vi "test Get-Set-Get Parameter Definitions.vi"(8 "error in":errorcluster, 11 "TestCase in":refnum<class "Scripting.lvclass">) -> (0 "error out":errorcluster, 3 "TestCase out":refnum<class "Scripting.lvclass">)   [LabVIEW 2020, in "Scripting.lvclass"]
uses:
  Scripting.lvclass
  Shared/Parameter Definition.ctl
  <vilib>/NI/NI VeriStand Encoding and Decoding/Encoding.ctl
  Scripting.lvclass/Scripting.ctl
  Scripting/Ballard/Constants.vi
  <vilib>/NI VeriStand/Custom Device Tools/Custom Device Utility Library/NI VeriStand - Search for Item by GUID.vi
  <vilib>/addons/_JKI Toolkits/VI Tester/TestCase.llb/TestCase.lvclass
  Scripting/Ballard/Ballard ARINC 429 Scripting.lvlib
  Scripting/ARINC 429/ARINC 429 Scripting.lvlib
  <vilib>/NI/NI VeriStand Encoding and Decoding/Encoding and Decoding.lvlib
  <vilib>/NI VeriStand/Custom Device Tools/Custom Device Utility Library/Custom Device Utility Library.lvlib
  <vilib>/NI VeriStand/Custom Device API/Custom Device API.lvlib
  C:/Program Files (x86)/National Instruments/LabVIEW 2020/vi.lib/addons/_JKI Toolkits/VI Tester/TestCase.llb/TestCase.lvclass
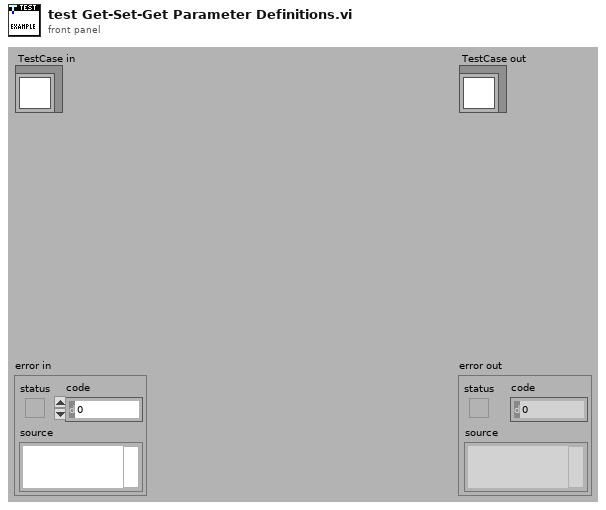
[diagram p1: front panel]
types:
  T1 = typedef "Parameter Definition.ctl" = cluster{"start index":i32, "size":i32, "encoding":T2, "signed":bool, "scale multiplier":dbl, "scale offset":dbl}
  T2 = typedef "Encoding and Decoding.lvlib/Encoding.ctl" = enum16{"BNR", "BCD", "Discrete"}
  T3 = typedef "Custom Device API.lvlib/Custom Device Item Ref.ctl" = u64
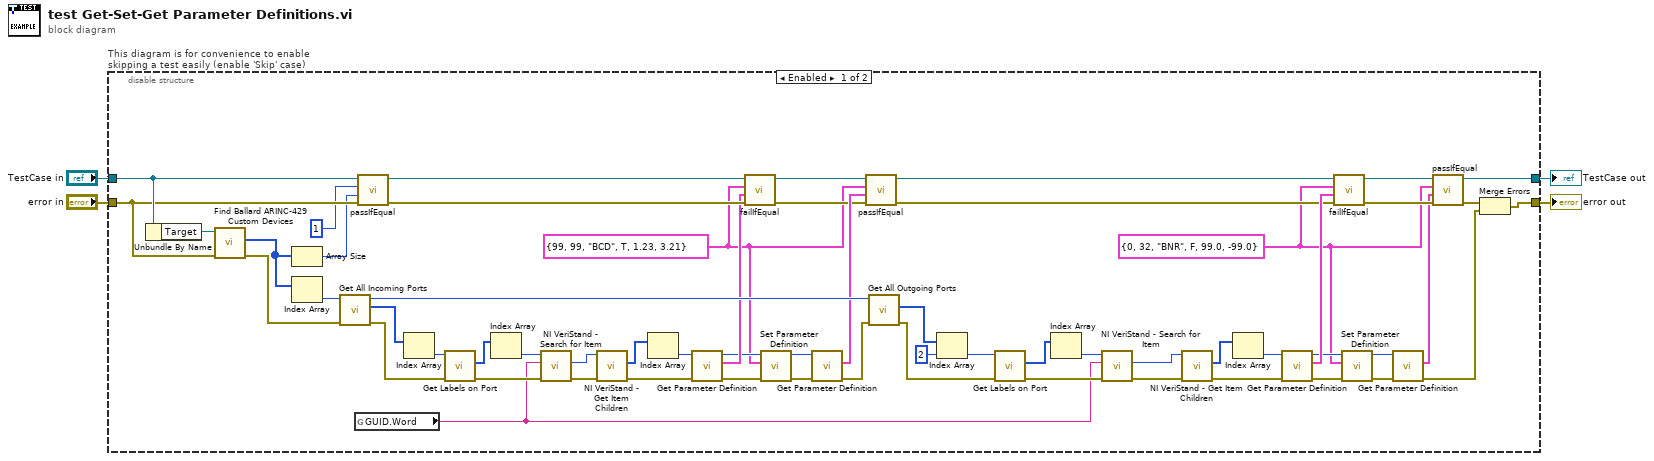
[diagram p0: block diagram]
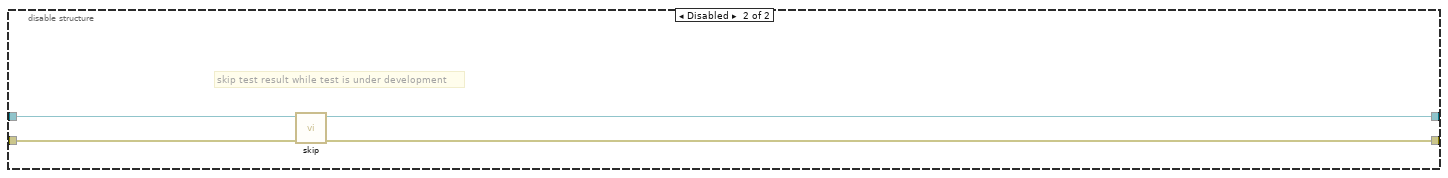
[diagram p2: hidden frame]
diagram:
  n1 = disable-structure "This diagram is for convenience to enable skipping a test easily (enable 'Skip' case)" shown="Enabled" {
    disable-tunnel: "TestCase in" -> [w62 w68]
    disable-tunnel: [w8 w66] -> w1
    disable-tunnel: [w51 w67] -> w3
    disable-tunnel: "error in" -> [w61 w65]
    frame Enabled {
      w17 = T1 {"start index"=99, "size"=99, "encoding"=enum."BCD", "signed"=TRUE, "scale multiplier"=1.23, "scale offset"=3.21} ("parameter definition")
      w6 = T1 {"start index"=0, "size"=32, "encoding"=enum."BNR", "signed"=FALSE, "scale multiplier"=99.0, "scale offset"=-99.0} ("parameter definition")
      n2 = Unbundle By Name(w62) -> ("Target"=w64:refnum<k24>)
      n3 = call "Find Ballard ARINC-429 Custom Devices.vi"("error in"=w61, "target in"=w64) -> ("error out"=w55:errorcluster, "Ballard ARINC 429 custom devices"=w5:u64[])  [unwired: 7 in, 1 out]
      n4 = Array Size(array=w5) -> (size(s)=w59:i32)
      n5 = Index Array(array=w5) -> (element=w63:u64)  [unwired: 1 in]
      n6 = call "Get All Incoming Ports.vi"("error in"=w55, "Ballard ARINC 429 custom device in"=w63) -> ("error out"=w48:errorcluster, "incoming ports"=w58:T3[], "Ballard ARINC 429 custom device out"=w54:T3)  [unwired: 7 in]
      n7 = global read "Constants.vi" "GUID.Word"() -> (w28:string)
      n8 = call-dynamic "passIfEqual.vi"("error in (no error)"=w61, "y"=w59, "x"=1 ("size(s)"), "TestCase in"=w62) -> ("error out"=w56:errorcluster, "TestCase out"=w57:refnum<class "Scripting.lvclass">)  [unwired: 6 in]
      n9 = Index Array(array=w58) -> (element=w49:T3)  [unwired: 1 in]
      n10 = call "Get Labels on Port.vi"("error in"=w48, "port in"=w49) -> ("error out"=w29:errorcluster, "labels"=w31:T3[])  [unwired: 6 in, 2 out]
      n11 = Index Array(array=w31) -> (element=w30:T3)  [unwired: 1 in]
      n12 = call-poly <vilib>:"NI VeriStand - Search for Item.vi"("error in"=w29, "Item GUID"=w28, "Section Ref in"=w30) -> ("error out"=w36:errorcluster, "Item Ref"=w35:T3)  [unwired: 5 in, 2 out]
      n13 = call <vilib>:"NI VeriStand - Get Item Children.vi"("error in (no error)"=w36, "Item Ref in"=w35) -> ("error out"=w33:errorcluster, "Child Refs"=w37:T3[])  [unwired: 6 in, 2 out]
      n14 = Index Array(array=w37) -> (element=w34:T3)  [unwired: 1 in]
      n15 = call "Get Parameter Definition.vi"("error in"=w33, "parameter ref in"=w34) -> ("error out"=w27:errorcluster, "parameter definition"=w32:T1, "parameter ref out"=w26:T3)  [unwired: 7 in]
      n16 = call-dynamic "failIfEqual.vi"("error in (no error)"=w56, "y"=w32, "x"=w17, "TestCase in"=w57) -> ("error out"=w21:errorcluster, "TestCase out"=w20:refnum<class "Scripting.lvclass">)  [unwired: 6 in]
      n17 = call "Set Parameter Definition.vi"("error in"=w27, "parameter definition"=w17, "parameter ref in"=w26) -> ("error out"=w25:errorcluster, "parameter ref out"=w24:T3)  [unwired: 7 in]
      n18 = call "Get Parameter Definition.vi"("error in"=w25, "parameter ref in"=w24) -> ("error out"=w23:errorcluster, "parameter definition"=w22:T1)  [unwired: 7 in, 1 out]
      n19 = call-dynamic "passIfEqual.vi"("error in (no error)"=w21, "y"=w22, "x"=w17, "TestCase in"=w20) -> ("error out"=w19:errorcluster, "TestCase out"=w18:refnum<class "Scripting.lvclass">)  [unwired: 6 in]
      n20 = call "Get All Outgoing Ports.vi"("error in"=w23, "Ballard ARINC 429 custom device in"=w54) -> ("error out"=w47:errorcluster, "outgoing ports"=w53:T3[])  [unwired: 7 in, 1 out]
      n21 = Index Array(array=w53, index=2) -> (element=w46:T3)
      n22 = call "Get Labels on Port.vi"("error in"=w47, "port in"=w46) -> ("error out"=w43:errorcluster, "labels"=w45:T3[])  [unwired: 6 in, 2 out]
      n23 = Index Array(array=w45) -> (element=w44:T3)  [unwired: 1 in]
      n24 = call-poly <vilib>:"NI VeriStand - Search for Item.vi"("error in"=w43, "Item GUID"=w28, "Section Ref in"=w44) -> ("error out"=w41:errorcluster, "Item Ref"=w42:T3)  [unwired: 5 in, 2 out]
      n25 = call <vilib>:"NI VeriStand - Get Item Children.vi"("error in (no error)"=w41, "Item Ref in"=w42) -> ("error out"=w40:errorcluster, "Child Refs"=w38:T3[])  [unwired: 6 in, 2 out]
      n26 = Index Array(array=w38) -> (element=w39:T3)  [unwired: 1 in]
      n27 = call "Get Parameter Definition.vi"("error in"=w40, "parameter ref in"=w39) -> ("error out"=w14:errorcluster, "parameter definition"=w50:T1, "parameter ref out"=w13:T3)  [unwired: 7 in]
      n28 = call-dynamic "failIfEqual.vi"("error in (no error)"=w19, "y"=w50, "x"=w6, "TestCase in"=w18) -> ("error out"=w11:errorcluster, "TestCase out"=w9:refnum<class "Scripting.lvclass">)  [unwired: 6 in]
      n29 = call "Set Parameter Definition.vi"("error in"=w14, "parameter definition"=w6, "parameter ref in"=w13) -> ("error out"=w15:errorcluster, "parameter ref out"=w16:T3)  [unwired: 7 in]
      n30 = call "Get Parameter Definition.vi"("error in"=w15, "parameter ref in"=w16) -> ("error out"=w12:errorcluster, "parameter definition"=w7:T1)  [unwired: 7 in, 1 out]
      n31 = call-dynamic "passIfEqual.vi"("error in (no error)"=w11, "y"=w7, "x"=w6, "TestCase in"=w9) -> ("error out"=w10:errorcluster, "TestCase out"=w8:refnum<class "Scripting.lvclass">)  [unwired: 6 in]
      n32 = Merge Errors(w10, w12) -> (w51:errorcluster)
    }
    frame Disabled {
      # "skip test result while test is under development"
      n33 = call <vilib>:"skip.vi"("error in (no error)"=w65, "TestCase in"=w68) -> ("error out"=w67:errorcluster, "TestCase out"=w66:refnum<class "Scripting.lvclass">)  [unwired: 8 in]
    }
  }
  "error out" <- w3
  "TestCase out" <- w1
